vi "Sort Funnels and Paths.vi"(8 "error in (no error)":errorcluster, 11 "Tool Data in":refnum<class "Tool Data.lvclass">) -> (0 "error out":errorcluster, 3 "Tool Data out":refnum<class "Tool Data.lvclass">)   [LabVIEW 2019, in "Tool Data.lvclass"]
uses:
  Tool Data.lvclass
  Tool Data.lvclass/Tool Data.ctl
  Parse/ParsePaths/Path.lvclass/Path.ctl
  Parse/ParsePaths/Path.lvclass
  Parse/PathCommands/PathCommands.lvclass
  Tool Object/Tool Object.lvclass
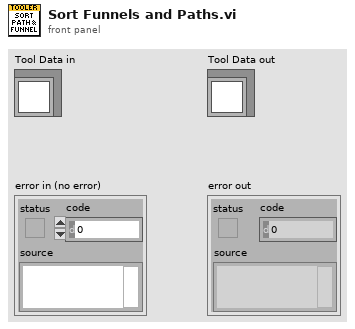
[diagram p1: front panel]
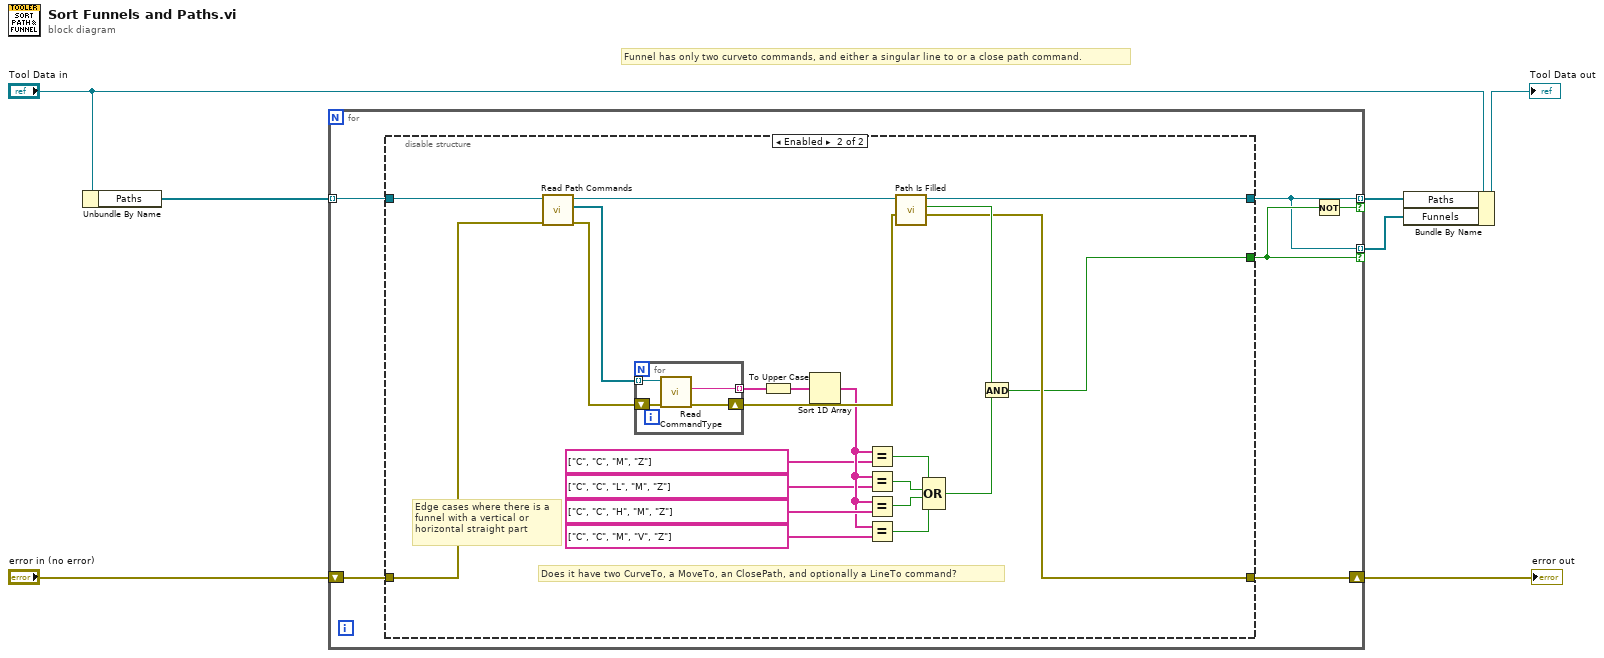
[diagram p0: block diagram]
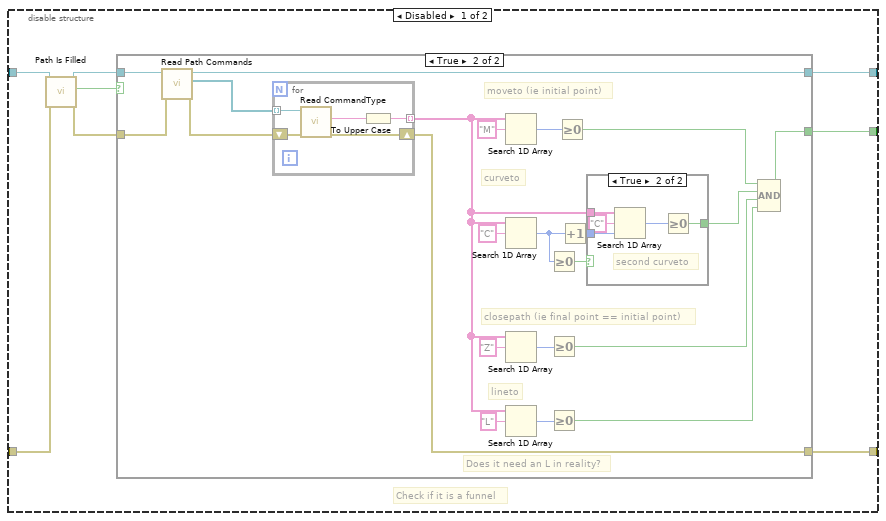
[diagram p2: hidden frame]
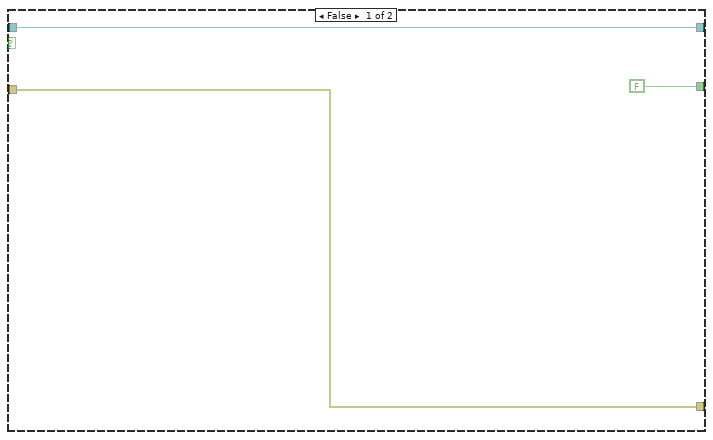
[diagram p3: hidden frame]
diagram:
  # "Funnel has only two curveto commands, and either a singular line to or a close path command."
  n1 = Unbundle By Name("Tool Data in") -> ("Paths"=w7:refnum<class "Path.lvclass">[])
  n2 = for {
    tunnel: w7 -> [w10] mode=indexing
    tunnel: [w11] -> w4 mode=indexing if=w13
    tunnel: [w11] -> w1 mode=indexing if=w12
    shift-right: [w8] -> w5
    shift-left: "error in (no error)" -> [w9]
    n3 = disable-structure shown="Enabled" {
      disable-tunnel: [w21 w68] -> w12
      disable-tunnel: [w20 w73] -> w11
      disable-tunnel: w10 -> [w17 w75]
      disable-tunnel: w9 -> [w15 w72]
      disable-tunnel: [w14 w69] -> w8
      frame Disabled {
        # "Check if it is a funnel"
        n4 = call "Path Is Filled.vi"("error in (no error)"=w15, "Path in"=w17) -> ("error out"=w16:errorcluster, "x != y?"=w19:bool, "Path out"=w18:refnum<class "Path.lvclass">)  [unwired: 7 in]
        n5 = case shown="True" w19 {
          tunnel: [FALSE w31] -> w21
          tunnel: w18 -> [w24 w30]
          tunnel: [w24 w29] -> w20
          tunnel: w16 -> [w22 w26]
          tunnel: [w22 w25] -> w14
          frame False {
          }
          frame True {
            # "Does it need an L in reality?"
            # "lineto"
            # "closepath (ie final point == initial point)"
            # "curveto"
            # "moveto (ie initial point)"
            n6 = call "Read Path Commands.vi"("error in (no error)"=w26, "Path in"=w30) -> ("error out"=w27:errorcluster, "Path Commands"=w28:refnum<class "PathCommands.lvclass">[], "Path out"=w29:refnum<class "Path.lvclass">)  [unwired: 7 in]
            n7 = for {
              tunnel: w28 -> [w57] mode=indexing
              tunnel: [w55] -> w32 mode=indexing
              shift-right: [w53] -> w25
              shift-left: w27 -> [w54]
              n8 = call-dynamic "Read CommandType.vi"("error in (no error)"=w54, "PathCommands in"=w57) -> ("error out"=w53:errorcluster, "CommandType"=w56:string)  [unwired: 7 in, 1 out]
              n9 = To Upper Case(1:w56) -> (0:w55:string)
            }
            n10 = Search 1D Array(1D array=w32, element="M") -> (index of element=w44:i32)  [unwired: 1 in]
            n11 = Search 1D Array(1D array=w32, element="C") -> (index of element=w43:i32)  [unwired: 1 in]
            n12 = Search 1D Array(1D array=w32, element="Z") -> (index of element=w40:i32)  [unwired: 1 in]
            n13 = Search 1D Array(1D array=w32, element="L") -> (index of element=w35:i32)  [unwired: 1 in]
            n14 = Greater Or Equal To 0?(x=w43) -> (x >= 0?=w42:bool)
            n15 = Greater Or Equal To 0?(x=w40) -> (x >= 0?=w37:bool)
            n16 = Greater Or Equal To 0?(x=w35) -> (x >= 0?=w33:bool)
            n17 = Greater Or Equal To 0?(x=w44) -> (x >= 0?=w39:bool)
            n18 = Increment(x=w43) -> (x+1=w36:i32)
            n19 = case shown="True" w42 {
              selector: w42 -> [w47 _]
              tunnel: w36 -> [_ w52]
              tunnel: w32 -> [_ w51]
              tunnel: [w47 w49] -> w38
              frame False {
              }
              frame True {
                # "second curveto"
                n20 = Search 1D Array(1D array=w51, element="C", start index (0)=w52) -> (index of element=w50:i32)
                n21 = Greater Or Equal To 0?(x=w50) -> (x >= 0?=w49:bool)
              }
            }
            n22 = Compound Arithmetic op=AND(w39, w38, w37, w33) -> (w31:bool)
          }
        }
      }
      frame Enabled {
        # "Edge cases where there is a funnel with a vertical or horizontal straight part"
        # "Does it have two CurveTo, a MoveTo, an ClosePath, and optionally a LineTo command?"
        n23 = call "Read Path Commands.vi"("error in (no error)"=w72, "Path in"=w75) -> ("error out"=w71:errorcluster, "Path Commands"=w79:refnum<class "PathCommands.lvclass">[], "Path out"=w74:refnum<class "Path.lvclass">)  [unwired: 7 in]
        n24 = for {
          tunnel: w79 -> [w83] mode=indexing
          tunnel: [w82] -> w78 mode=indexing
          shift-right: [w80] -> w70
          shift-left: w71 -> [w81]
          n25 = call-dynamic "Read CommandType.vi"("error in (no error)"=w81, "PathCommands in"=w83) -> ("error out"=w80:errorcluster, "CommandType"=w82:string)  [unwired: 7 in, 1 out]
        }
        n26 = To Upper Case(1:w78) -> (0:w77:string[])
        n27 = Sort 1D Array(array=w77) -> (sorted array=w65:string[])
        n28 = Equal?(x=w65, y=string[] ["C", "C", "M", "Z"] ("sorted array")) -> (x = y?=w64:bool)
        n29 = Equal?(x=w65, y=string[] ["C", "C", "L", "M", "Z"] ("sorted array")) -> (x = y?=w59:bool)
        n30 = Equal?(x=w65, y=string[] ["C", "C", "H", "M", "Z"] ("sorted array")) -> (x = y?=w58:bool)
        n31 = Equal?(x=w65, y=string[] ["C", "C", "M", "V", "Z"] ("sorted array")) -> (x = y?=w63:bool)
        n32 = call "Path Is Filled.vi"("error in (no error)"=w70, "Path in"=w74) -> ("error out"=w69:errorcluster, "x != y?"=w76:bool, "Path out"=w73:refnum<class "Path.lvclass">)  [unwired: 7 in]
        n33 = Compound Arithmetic op=OR(w64, w59, w58, w63) -> (w62:bool)
        n34 = And(x=w76, y=w62) -> (x .and. y?=w68:bool)
      }
    }
    n35 = Not(x=w12) -> (.not. x?=w13:bool)
  }
  "error out" <- w5
  n36 = Bundle By Name(cluster="Tool Data in", "Paths"=w4, "Funnels"=w1) -> (→"Tool Data out":refnum<class "Tool Data.lvclass">)
